vi "Module Loop.vi"(8 "error in (no error)":errorcluster, 11 "Config Alert Module in":refnum<class "Config Monitor Module.lvclass">) -> (0 "error out":errorcluster, 3 "Config Alert Module out":refnum<class "Config Monitor Module.lvclass">)   [LabVIEW 2020, in "VolatusGUI.lvlib" / "Config Monitor Module.lvclass"]
uses:
  Config Monitor Module.lvclass
  C:/dev/lv20CE/relink/lv-volatus/Volatus/Module/Module.lvclass
  Node Config Info.ctl
  Module/Module.lvclass/Module.ctl
  MessageQ/MessageQ.lvclass/MessageQ.ctl
  Module/Module.lvclass
  Config Monitor Module.lvclass/Config Monitor Module.ctl
  <vilib>/Utility/error.llb/Error Cluster From Error Code.vi
  lv-promises/Promises/Promise/Promise.lvclass
  MessageQ/MessageQ.lvclass
  System Config Status API/System Config Status API.lvclass
  VolatusGUI/GUI Helper/GUI Helper.lvclass
  C:/dev/lv20CE/relink/lv-volatus/Volatus/Config Alert Module/Config Monitor Module.lvclass
  Volatus.lvlib
panel:
  in  "Update Config":bool
  in  "Load Config":bool
  in  "Reload Config":bool
  out "Config Hash":string
  out "Config Version":string
  in  "Array":T1[](array[typedef])
  # "This Node"
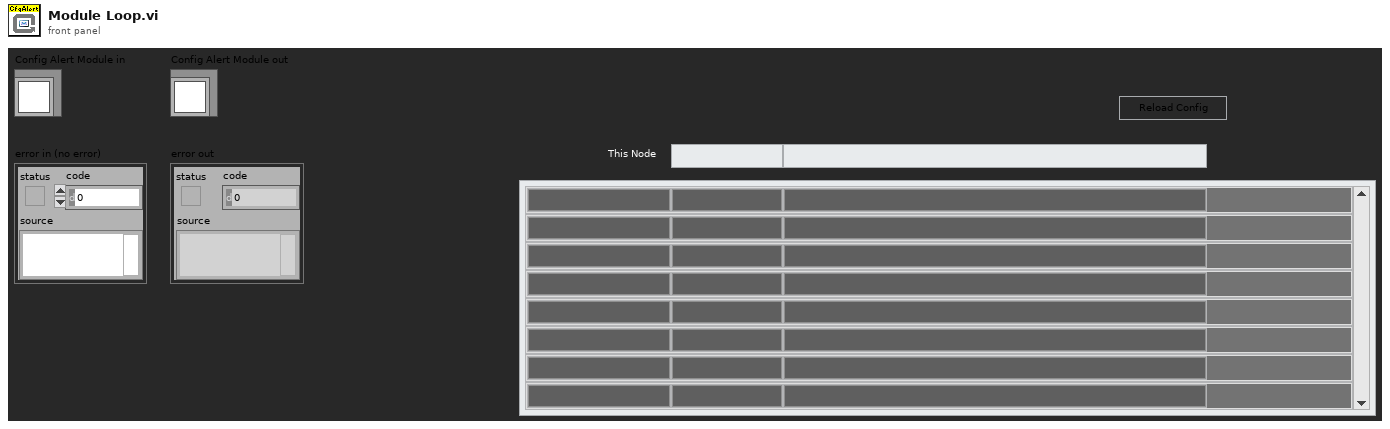
[diagram p1: front panel]
types:
  T1 = typedef "Volatus.lvlib/Node Config Info.ctl" = cluster{"Node":string, "Config Version":string, "Config Hash":string, "Pull":bool, "Push":bool, "Version Color":u32, "Hash Color":u32, "Node Color":u32}
  T2 = enum32{"Invalid", "Standard", "Closed", "Hidden", "Minimized", "Maximized"}
  T3 = cluster{"Node":bool, "Config Version":bool, "Config Hash":bool, "Pull":bool, "Push":bool, "Version Color":bool, "Hash Color":bool, "Node Color":bool}[]
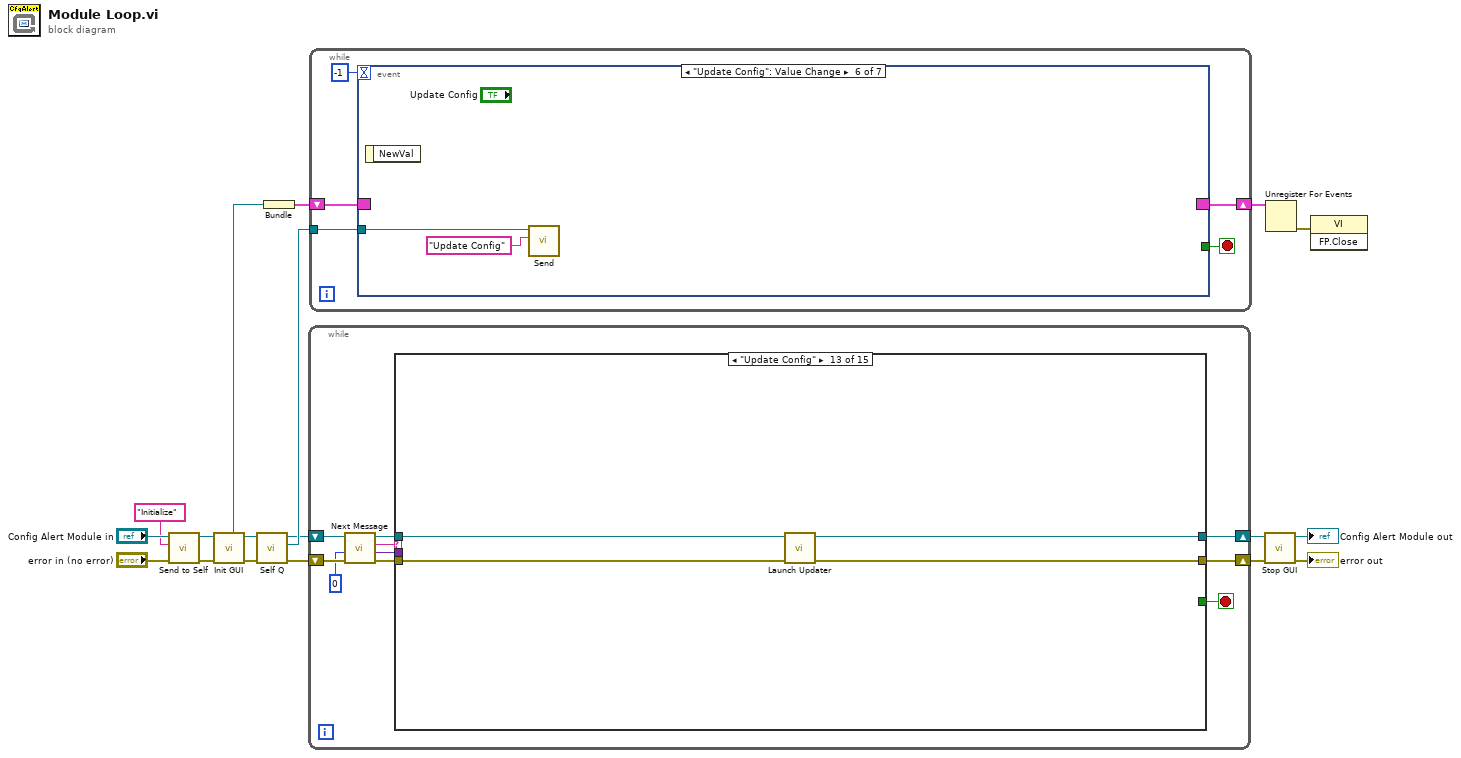
[diagram p0: block diagram]
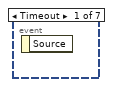
[diagram p2: hidden frame]
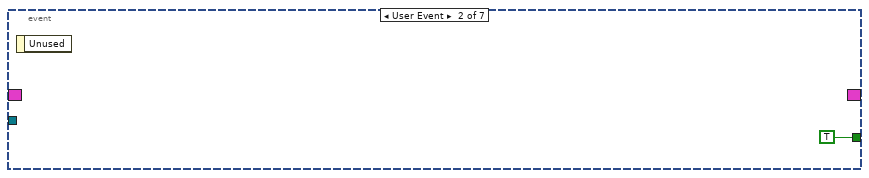
[diagram p3: hidden frame]
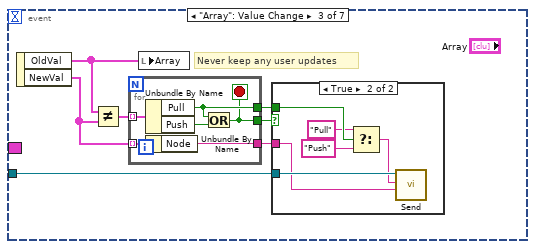
[diagram p4: hidden frame]
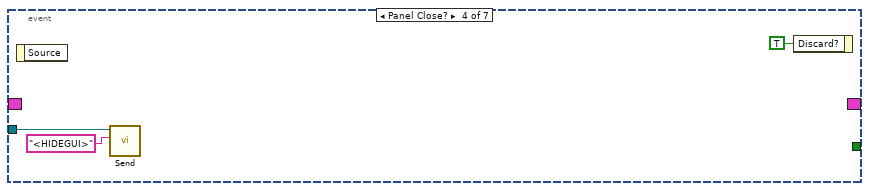
[diagram p6: hidden frame]
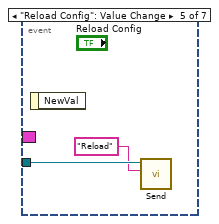
[diagram p7: hidden frame]
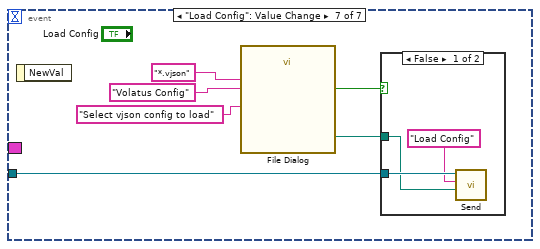
[diagram p8: hidden frame]
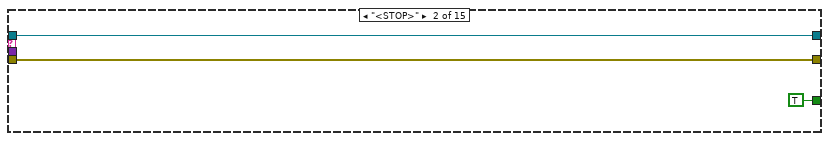
[diagram p11: hidden frame]
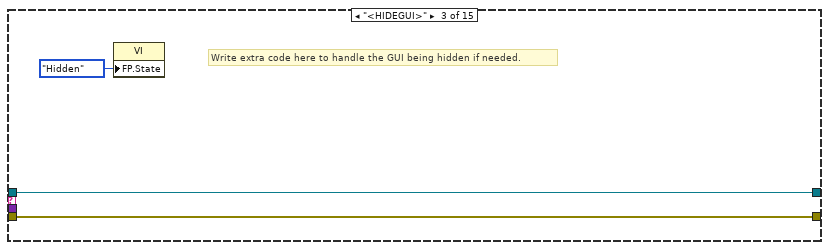
[diagram p12: hidden frame]
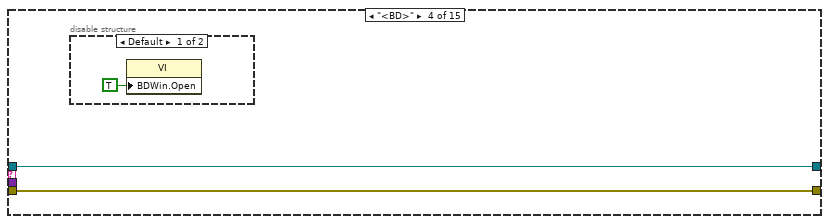
[diagram p13: hidden frame]
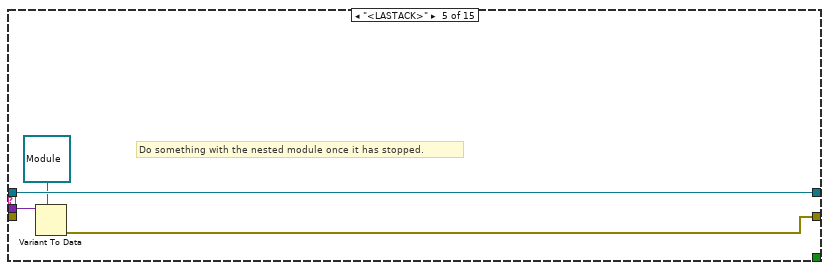
[diagram p15: hidden frame]
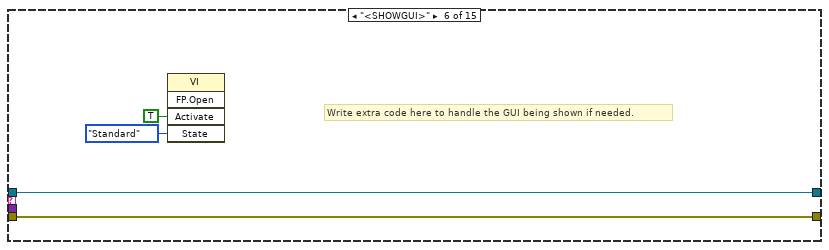
[diagram p16: hidden frame]
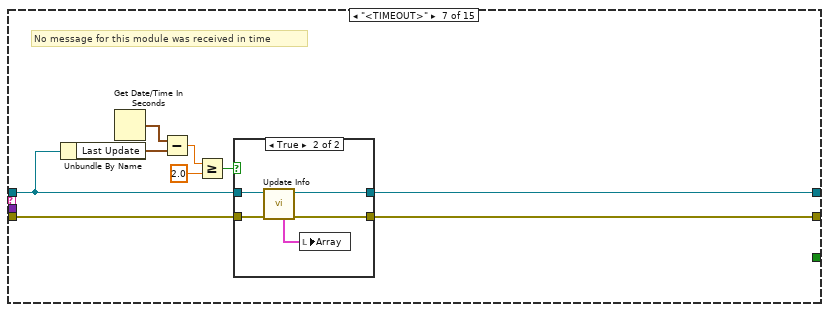
[diagram p17: hidden frame]
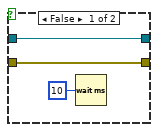
[diagram p18: hidden frame]
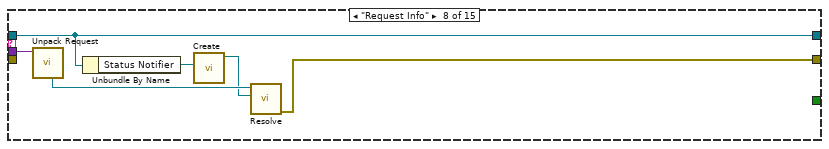
[diagram p19: hidden frame]
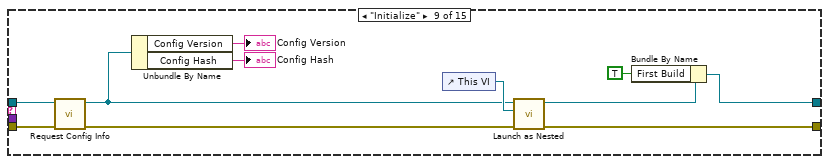
[diagram p20: hidden frame]
diagram:
  n1 = call "Send to Self.vi"("error in (no error)"="error in (no error)", "Message ID"="Initialize", "Module in"="Config Alert Module in") -> ("error out"=w4:errorcluster, "Module out"=w2:refnum<class "Config Monitor Module.lvclass">)  [unwired: 7 in]
  n2 = call "Init GUI.vi"("Module in"=w2) -> ("Module in"=w10:refnum<class "Config Monitor Module.lvclass">, "Event Reg"=w15:refnum<event-registration>)  [unwired: 9 in]
  n3 = call "Self Q.vi"("Module in"=w10) -> ("Self Q"=w9:refnum<class "MessageQ.lvclass">, "Module in"=w8:refnum<class "Config Monitor Module.lvclass">)  [unwired: 9 in]
  n4 = Bundle("Event Reg"=w15) -> (w11:cluster{"Event Reg":refnum<event-registration>})  [unwired: 1 in]
  n5 = while {
    shift-right: [w21] -> w13
    shift-left: w8 -> [w26]
    shift-right: [w20] -> w14
    shift-left: w4 -> [w25]
    stop <- w19 stop-if-true
    n6 = call "Next Message.vi"("error in (no error)"=w25, "Timeout ms (-1)"=0, "Module in"=w26) -> ("error out"=w24:errorcluster, "Data"=w18:variant, "ID"=w23:string, "Module in"=w22:refnum<class "Config Monitor Module.lvclass">)  [unwired: 5 in]
    n7 = case shown="\"Update Config\"" w23 {
      tunnel: w24 -> [w27 w30 w33 w35 _ w44 w54 _ w79 _ _ _ w125 _ w147]
      tunnel: w22 -> [w28 w31 w34 w36 w41 w45 w51 w65 w70 w84 w104 w120 w123 w135 w145]
      tunnel: [w28 w31 w34 w36 w41 w45 w52 w65 w76 w82 w99 w120 w122 w129 w144] -> w21
      tunnel: [w27 w30 w33 w35 w38 w44 w53 w66 w74 w81 w100 w121 w124 w128 w146] -> w20
      tunnel: [_ TRUE _ _ _ _ _ _ _ _ _ _ _ _ _] -> w19
      tunnel: w18 -> [_ _ _ _ w40 _ _ w68 _ w90 w109 _ _ w134 _]
      frame "<CLOSE>" {
        # "If the module might be in a state that can be stopped, add logic to decide whether or not to actually stop."
        # "Add additional code to handle stopping the module."
      }
      frame "<STOP>" {
      }
      frame "<HIDEGUI>" {
        # "Write extra code here to handle the GUI being hidden if needed."
        n8 = property class="VI"("FP.State"=T2."Hidden" ("Front Panel Window:State")) -> ()  [unwired: 2 in, 2 out]
      }
      frame "<BD>" {
        n9 = disable-structure shown="Default" {
          frame condition #0 (active) {
            n10 = property class="VI"("BDWin.Open"=TRUE ("Block Diagram Window:Open")) -> ()  [unwired: 2 in, 2 out]
          }
          frame condition #1 {
          }
        }
      }
      frame "<LASTACK>" {
        # "Do something with the nested module once it has stopped."
        n11 = Variant To Data(type=refnum<class "Module.lvclass"> refnum ("Volatus:Module"), Variant=w40) -> (error out=w38:errorcluster)  [unwired: 1 in, 1 out]
      }
      frame "<SHOWGUI>" {
        # "Write extra code here to handle the GUI being shown if needed."
        n12 = invoke class="VI" method="FP.Open"("Activate"=TRUE ("Activate?"), "State"=T2."Standard") -> ()  [unwired: 3 in, 5 out]
      }
      frame "<TIMEOUT>" {
        # "No message for this module was received in time"
        n13 = Unbundle By Name(w51) -> ("Last Update"=w49:timestamp)
        n14 = Get Date/Time In Seconds() -> (seconds since 1Jan1904=w50:timestamp)
        n15 = Subtract(x=w50, y=w49) -> (x-y=w48:dbl)
        n16 = Greater Or Equal?(x=w48, y=2.0) -> (x >= y?=w46:bool)
        n17 = case shown="True" w46 {
          tunnel: w54 -> [w56 w62]
          tunnel: [w56 w60] -> w53
          tunnel: [w57 w59] -> w52
          tunnel: w51 -> [w57 w58]
          frame False {
            n18 = Wait (ms)(milliseconds to wait=u32 10) -> ()  [unwired: 1 out]
          }
          frame True {
            n19 = call "Update Info.vi"("error in (no error)"=w62, "Config Monitor Module in"=w58) -> ("error out"=w60:errorcluster, "Config Monitor Module out"=w59:refnum<class "Config Monitor Module.lvclass">, "Node Config Info"=w61:T1[])  [unwired: 7 in]
            n20 = local write "Array"(w61) -> ()
          }
        }
      }
      frame "Request Info" {
        n21 = call "Unpack Request.vi"("Request Data"=w68) -> ("Promise"=w67:refnum<class "Promise.lvclass">)  [unwired: 8 in, 2 out]
        n22 = Unbundle By Name(w65) -> ("Status Notifier"=w64:refnum<notifier>)
        n23 = call "Create.vi"("Status Notifier"=w64) -> ("System Config Status API out"=w63:refnum<class "System Config Status API.lvclass">)  [unwired: 10 in]
        n24 = call "Resolve.vi"("Result (None)"=w63, "Promise in"=w67) -> ("error out"=w66:errorcluster)  [unwired: 8 in, 1 out]
      }
      frame "Initialize" {
        n25 = call "Request Config Info.vi"("error in (no error)"=w79, "Config Monitor Module in"=w70) -> ("error out"=w71:errorcluster, "Config Monitor Module out"=w69:refnum<class "Config Monitor Module.lvclass">)  [unwired: 8 in]
        n26 = Unbundle By Name(w69) -> ("Config Version"=→"Config Version":string, "Config Hash"=→"Config Hash":string)
        n27 = control-ref of="This VI"() -> (w72:refnum<vi>)
        n28 = call "Launch as Nested.vi"("error in (no error)"=w71, "GUI"=w72, "Parent in"=w69) -> ("error out"=w74:errorcluster, "Parent in"=w73:refnum<class "Config Monitor Module.lvclass">)  [unwired: 6 in, 1 out]
        n29 = Bundle By Name(cluster=w73, "First Build"=TRUE) -> (w76:refnum<class "Config Monitor Module.lvclass">)
      }
      frame "Push" {
        n30 = Variant To Data(type="", Variant=w90) -> (data=w80:string, error out=w83:errorcluster)  [unwired: 1 in]
        n31 = Format Into String(format string="This will deploy the local config to \"%s\" and then the remote system will reboot.\nDo you want to continue?", w80) -> (resulting string=w87:string)  [unwired: 2 in, 1 out]
        n32 = Two Button Dialog(message=w87, 2:"Push Config" ("T button name (\"OK\")")) -> (T button?=w85:bool)  [unwired: 1 in]
        n33 = case shown="True" w85 {
          tunnel: w84 -> [w92 w98]
          tunnel: w83 -> [w91 w93]
          tunnel: [w92 w98] -> w82
          tunnel: [w91 w94] -> w81
          tunnel: w80 -> [_ w96]
          frame False {
          }
          frame True {
            n34 = Unbundle By Name(w98) -> ("Config Manager"=w97:refnum<class "MessageQ.lvclass">)
            n35 = call "Send.vi"("error in (no error)"=w93, "Data"=w96, "ID"="Push Config" ("Message ID"), "MessageQ in"=w97) -> ("error out"=w94:errorcluster)  [unwired: 6 in, 1 out]
          }
        }
      }
      frame "Pull" {
        n36 = Variant To Data(type="", Variant=w109) -> (data=w101:string, error out=w102:errorcluster)  [unwired: 1 in]
        n37 = Format Into String(format string="This will update the local config from the \"%s\" node and then the program will restart.\nDo you want to continue?", w101) -> (resulting string=w106:string)  [unwired: 2 in, 1 out]
        n38 = Two Button Dialog(message=w106, 2:"Pull Config" ("T button name (\"OK\")")) -> (T button?=w103:bool)  [unwired: 1 in]
        n39 = case shown="True" w103 {
          tunnel: w104 -> [w111 w117]
          tunnel: w102 -> [w110 w112]
          tunnel: [w111 w117] -> w99
          tunnel: [w110 w113] -> w100
          tunnel: w101 -> [_ w115]
          frame False {
          }
          frame True {
            n40 = Unbundle By Name(w117) -> ("Config Manager"=w116:refnum<class "MessageQ.lvclass">)
            n41 = call "Send.vi"("error in (no error)"=w112, "Data"=w115, "ID"="Pull Config" ("Message ID"), "MessageQ in"=w116) -> ("error out"=w113:errorcluster)  [unwired: 6 in, 1 out]
          }
        }
      }
      frame "Reload" {
        n42 = Unbundle By Name(w120) -> ("Config Manager"=w119:refnum<class "MessageQ.lvclass">)
        n43 = call "Send.vi"("ID"="Reload Config" ("Message ID"), "MessageQ in"=w119) -> ("error out"=w121:errorcluster)  [unwired: 8 in, 1 out]
      }
      frame "Update Config" {
        n44 = call "Launch Updater.vi"("error in (no error)"=w125, "Config Monitor Module in"=w123) -> ("error out"=w124:errorcluster, "Config Monitor Module out"=w122:refnum<class "Config Monitor Module.lvclass">)  [unwired: 8 in]
      }
      frame "Load Config" {
        n45 = Variant To Data(type=path "", Variant=w134) -> (data=w132:path, error out=w131:errorcluster)  [unwired: 1 in]
        n46 = Read from Binary File(8:w131, 10:-1 ("count (1)"), 11:w132) -> (0:w127:errorcluster, 2:w126:string)  [unwired: 3 in, 2 out]
        n47 = case shown="No Error" w127 {
          selector: w127 -> [w141 w142]
          tunnel: w135 -> [w138 w143]
          tunnel: [w138 w143] -> w129
          tunnel: [w137 w142] -> w128
          tunnel: w126 -> [w136 _]
          frame No Error {
            n48 = Unbundle By Name(w138) -> ("Config Manager"=w140:refnum<class "MessageQ.lvclass">)
            n49 = call "Send.vi"("error in (no error)"=w141, "Data"=w136, "ID"="Update Config" ("Message ID"), "MessageQ in"=w140) -> ("error out"=w137:errorcluster)  [unwired: 6 in, 1 out]
          }
          frame Error {
          }
        }
      }
      frame Default {
        n50 = call "Report Unhandled Message ID.vi"("error in (no error)"=w147, "Module in"=w145) -> ("error out"=w146:errorcluster, "Module in"=w144:refnum<class "Config Monitor Module.lvclass">)  [unwired: 8 in]
      }
    }
  }
  n51 = while {
    tunnel: w9 -> [w152]
    shift-right: [w150] -> w12
    shift-left: w11 -> [w151]
    stop <- w149 stop-if-true
    n52 = event shown="[5] \"Update Config\": Value Change" {
      selector: w151 -> [_ _ _ _ _ _ _]
      dyn-events: [_ _ _ _ _ _ _] -> w150
      timeout: -1 -> [_ _ _ _ _ _ _]
      tunnel: w152 -> [_ _ w156 w174 w177 w179 w180]
      tunnel: [_ TRUE _ _ _ _ _] -> w149
      event Timeout {
        n53 = event-data() -> ()  [unwired: 1 in, 1 out]
      }
      event User Event {
        n54 = event-data() -> ()  [unwired: 1 in, 1 out]
      }
      event "Array": Value Change {
        # "Never keep any user updates"
        n55 = event-data() -> ("OldVal"=w160:T1[], "NewVal"=w158:T1[])  [unwired: 1 in]
        n56 = Not Equal?(x=w160, y=w158) -> (x != y?=w159:T3)
        n57 = for {
          tunnel: w159 -> [w172] mode=indexing
          tunnel: w158 -> [w171] mode=indexing
          tunnel: [w169] -> w157
          tunnel: [w170] -> w154
          tunnel: [w167] -> w155
          stop <- w167 stop-if-true
          n58 = Unbundle By Name(w172) -> ("Pull"=w169:bool, "Push"=w168:bool)
          n59 = Unbundle By Name(w171) -> ("Node"=w170:string)
          n60 = Or(x=w169, y=w168) -> (x .or. y?=w167:bool)
        }
        n61 = local write "Array"(w160) -> ()
        n62 = case shown="True" w155 {
          tunnel: w157 -> [_ w166]
          tunnel: w156 -> [_ w163]
          tunnel: w154 -> [_ w161]
          frame False {
          }
          frame True {
            n63 = Select(t="Pull", s=w166, f="Push") -> (s? t:f=w162:string)
            n64 = call "Send.vi"("Data"=w161, "ID"=w162, "MessageQ in"=w163) -> ()  [unwired: 7 in, 2 out]
          }
        }
      }
      event Panel Close? {
        n65 = event-data() -> ()  [unwired: 1 in, 1 out]
        n66 = call "Send.vi"("ID"="<HIDEGUI>", "MessageQ in"=w174) -> ()  [unwired: 8 in, 2 out]
        n67 = event-data("Discard?"=TRUE) -> ()  [unwired: 1 in, 1 out]
      }
      event "Reload Config": Value Change {
        n68 = event-data() -> ()  [unwired: 1 in, 1 out]
        n69 = call "Send.vi"("ID"="Reload", "MessageQ in"=w177) -> ()  [unwired: 8 in, 2 out]
      }
      event "Update Config": Value Change {
        n70 = event-data() -> ()  [unwired: 1 in, 1 out]
        n71 = call "Send.vi"("ID"="Update Config", "MessageQ in"=w179) -> ()  [unwired: 8 in, 2 out]
      }
      event "Load Config": Value Change {
        n72 = event-data() -> ()  [unwired: 1 in, 1 out]
        n73 = call "File Dialog"("prompt"="Select vjson config to load", "pattern (all files)"="*.vjson", "pattern label"="Volatus Config") -> ("selected path"=w181:path, "cancelled"=w182:bool)  [unwired: 9 in, 2 out]
        n74 = case shown="False" w182 {
          tunnel: w181 -> [w186 _]
          tunnel: w180 -> [w188 _]
          frame False {
            n75 = call "Send.vi"("Data"=w186, "ID"="Load Config", "MessageQ in"=w188) -> ()  [unwired: 7 in, 2 out]
          }
          frame True {
          }
        }
      }
    }
  }
  n76 = call "Stop GUI.vi"("error in (no error)"=w14, "Module in"=w13) -> ("error out"=→"error out":errorcluster, "Module in"=→"Config Alert Module out":refnum<class "Config Monitor Module.lvclass">)  [unwired: 8 in]
  n77 = Unregister For Events(event registration refnum=w12) -> (error out=w16:errorcluster)  [unwired: 1 in]
  n78 = invoke class="VI" method="FP.Close"(error in=w16) -> ()  [unwired: 2 in, 3 out]
